vi "Wrap Pinmap.vi"(8 "error in":errorcluster, 10 "DUT pin":string, 11 "measurement context in":refnum<class "Measure Call Context.lvclass">) -> (0 "error out":errorcluster, 1 "Channel":string, 2 "session reservation out":refnum<class "Session Reservation.lvclass">, 3 "measurement context out":refnum<class "Measure Call Context.lvclass">)   [LabVIEW 2025, in "Automotive Vision.lvclass"]
uses:
  Automotive Vision.lvclass
  <vilib>/Plug-In SDKs/Measurements/Measure Call Context/Measure Call Context.lvclass
  <vilib>/Plug-In SDKs/Clients/Session Management V1/Session Reservation/Session Reservation.lvclass
  <vilib>/Plug-In SDKs/Measurements/Measure Call Context/Reserve Sessions - 1Pin.vi
  session-management/flexrio148x/Session Management flexrio 148x.lvlib
  <vilib>/Plug-In SDKs/Clients/Session Management V1/Session Reservation/Initialize and Close Session Behavior.ctl
  <vilib>/Plug-In SDKs/Clients/Session Management V1/Session Reservation/Connection.ctl
  session-management/flexrio148x/Connection with Session.ctl
panel:
  out "connection":T1
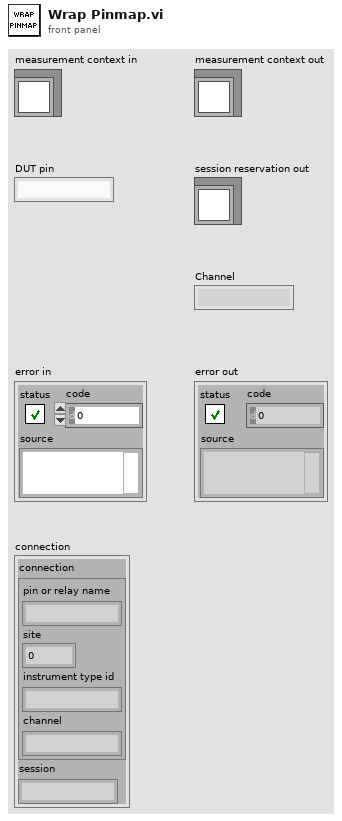
[diagram p1: front panel]
types:
  T1 = typedef "Session Management flexrio 148x.lvlib/Connection with Session.ctl" = cluster{"connection":T2, "session":string}
  T2 = typedef "NI Session Management V1 Client.lvlib/Session Reservation.lvclass/Connection.ctl" = cluster{"pin or relay name":string, "site":i32, "instrument type id":string, "channel":string}
  T3 = typedef "NI Session Management V1 Client.lvlib/Session Reservation.lvclass/Initialize and Close Session Behavior.ctl" = enum16{"Auto", "Initialize and Close", "Attach and Detach", "Initialize and Detach", "Attach and Close"}
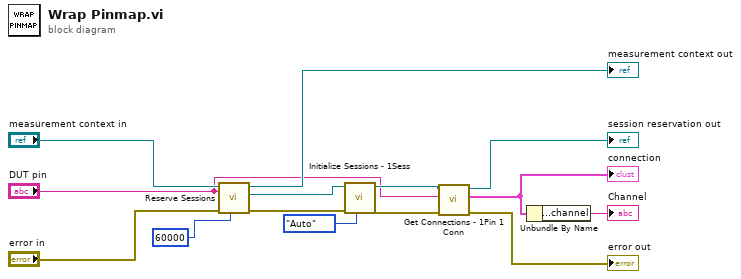
[diagram p0: block diagram]
diagram:
  n1 = call-poly <vilib>:"Reserve Sessions.vi"("timeout (ms)"=60000, "error in"="error in", "pin or relay name"="DUT pin", "measurement context in"="measurement context in") -> ("error out"=w11:errorcluster, "session reservation out"=w10:refnum<class "Session Reservation.lvclass">, "measurement context out"=→"measurement context out":refnum<class "Measure Call Context.lvclass">)  [unwired: 5 in]
  n2 = call "Initialize Sessions - 1Sess.vi"("initialize and close session behavior"=Initialize_and_Close_Session_Behavior."Auto", "error in"=w11, "session reservation in"=w10) -> ("error out"=w8:errorcluster, "session reservation out"=w6:refnum<class "Session Reservation.lvclass">)  [unwired: 5 in, 2 out]
  n3 = call "Get Connections - 1Pin 1 Conn.vi"("error in"=w8, "pin or relay name"="DUT pin", "session reservation in"=w6) -> ("error out"=→"error out":errorcluster, "connection"=w4:T1, "session reservation out"=→"session reservation out":refnum<class "Session Reservation.lvclass">)  [unwired: 6 in]
  "connection" <- w4
  n4 = Unbundle By Name(w4) -> ("connection.channel"=→"Channel":string)
